vi "Add Bitfile Dialog.vi"(8 "error in (no error)":errorcluster, 11 "Item Ref in":T1 format="%.0x") -> (0 "error out":errorcluster, 1 "RIO Device Address out":string, 2 "Bitfile Path out":path, 3 "Item Ref out":T1 format="%.0x", 5 "OK?":bool)   [LabVIEW 2020, in "Engine Simulation Toolkit System Explorer.lvlib"]
uses:
  Engine Simulation Toolkit System Explorer.lvlib
  <vilib>/NI VeriStand/Custom Device API/Custom Device Item Ref.ctl
  Shared/Properties.vi
  <vilib>/NI VeriStand/Custom Device API/Get Item Property (String Array).vi
  <vilib>/NI VeriStand/Custom Device API/Custom Device API.lvlib
  Shared/Engine Simulation Toolkit Shared.lvlib
panel:
  in  "Warning text":string
  in  "Cancel":bool
  in  "OK":bool
  in  "RIO Device Address":string="RIO0"
  in  "Bitfile Path":path
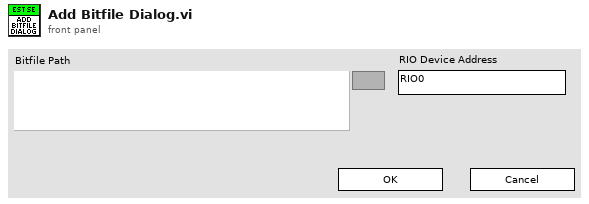
[diagram p1: front panel]
types:
  T1 = typedef "Custom Device API.lvlib/Custom Device Item Ref.ctl" = u64
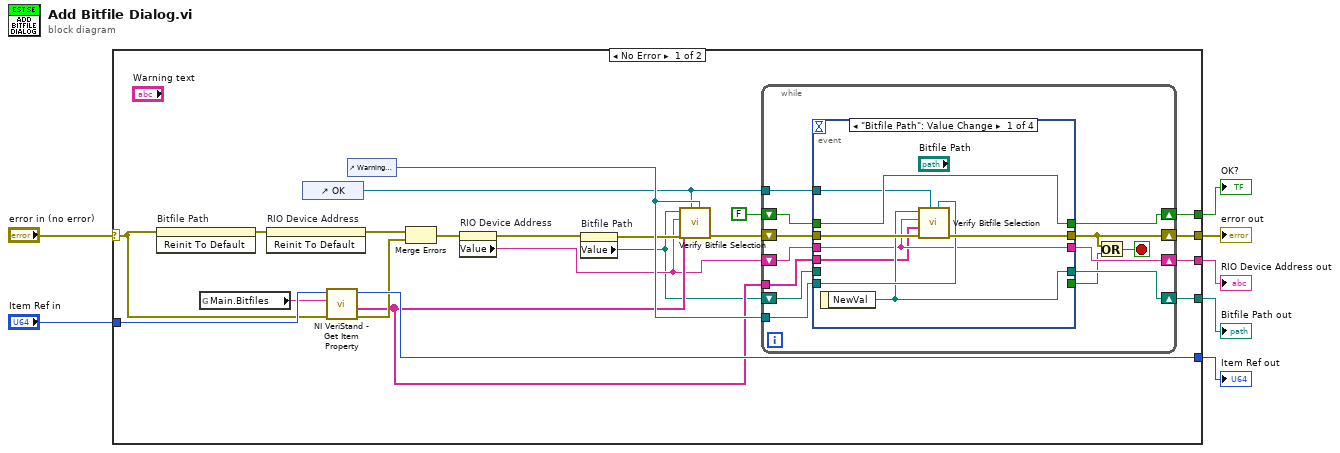
[diagram p0: block diagram]
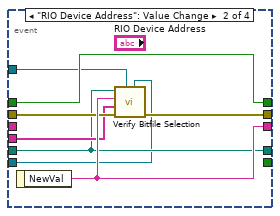
[diagram p2: hidden frame]
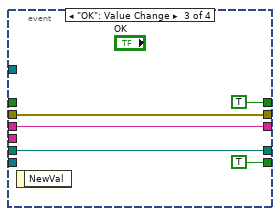
[diagram p3: hidden frame]
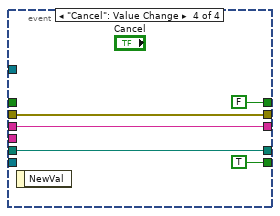
[diagram p4: hidden frame]
diagram:
  n1 = case shown="No Error" "error in (no error)" {
    selector: "error in (no error)" -> [w20 w69]
    tunnel: [w23 w69] -> w7
    tunnel: [w26 _] -> w5
    tunnel: [w25 _] -> w4
    tunnel: [w24 _] -> w3
    tunnel: "Item Ref in" -> [w22 w68]
    tunnel: [w21 w68] -> w1
    frame No Error {
      n2 = invoke on="Bitfile Path" class="Path" method="Reinit To Default"(error in=w20) -> (error out=w28:errorcluster)  [unwired: 2 in, 2 out]
      n3 = global read "Properties.vi" "Main.Bitfiles"() -> (w18:string)
      n4 = invoke on="RIO Device Address" class="Str" method="Reinit To Default"(error in=w28) -> (error out=w8:errorcluster)  [unwired: 2 in, 2 out]
      n5 = control-ref of="OK"() -> (w9:refnum<vi>)
      n6 = call-poly <vilib>:"NI VeriStand - Get Item Property.vi"("error in (no error)"=w20, "Property Name"=w18, "Item Ref in"=w22) -> ("error out"=w19:errorcluster, "Value"=w15:string[], "Item Ref out"=w21:T1)  [unwired: 5 in, 1 out]
      n7 = control-ref of="Warning text"() -> (w16:refnum<vi>)
      n8 = Merge Errors(w8, w19) -> (w14:errorcluster)
      n9 = property on="RIO Device Address" class="Str"(error in=w14) -> (error out=w13:errorcluster, "Value"=w11:string)  [unwired: 1 in, 1 out]
      n10 = property on="Bitfile Path" class="Path"(error in=w13) -> (error out=w12:errorcluster, "Value"=w10:path)  [unwired: 1 in, 1 out]
      n11 = call "Verify Bitfile Selection.vi"("Warning text reference"=w16, "ok button reference in"=w9, "error in (no error)"=w12, "Existing RIO Device Addresses"=w15, "RIO Device Address"=w11, "file path"=w10) -> ("error out"=w17:errorcluster)  [unwired: 5 in]
      n12 = while {
        shift-right: [w39] -> w26
        shift-left: w10 -> [w37]
        shift-right: [w40] -> w25
        shift-left: w11 -> [w38]
        shift-right: [w41] -> w24
        shift-left: FALSE -> [w36]
        tunnel: w9 -> [w35]
        shift-right: [w31] -> w23
        shift-left: w17 -> [w32]
        tunnel: w15 -> [w29]
        tunnel: w16 -> [w30]
        stop <- w34 stop-if-true
        n13 = event shown="[0] \"Bitfile Path\": Value Change" {
          selector: _ -> [_ _ _ _]
          dyn-events: _ -> [_ _ _ _]
          timeout: _ -> [_ _ _ _]
          tunnel: [_ _ TRUE TRUE] -> w33
          tunnel: [w43 w56 w59 w65] -> w40
          tunnel: [w44 w52 w60 w64] -> w39
          tunnel: [w49 w57 TRUE FALSE] -> w41
          tunnel: w38 -> [w43 _ w59 w65]
          tunnel: w37 -> [_ w52 w60 w64]
          tunnel: w36 -> [w49 w57 _ _]
          tunnel: w35 -> [w46 w51 _ _]
          tunnel: w32 -> [w48 w55 w58 w63]
          tunnel: [w47 w54 w58 w63] -> w31
          tunnel: w30 -> [w45 w50 _ _]
          tunnel: w29 -> [w42 w53 _ _]
          event "Bitfile Path": Value Change {
            n14 = event-data() -> ("NewVal"=w44:path)  [unwired: 1 in]
            n15 = call "Verify Bitfile Selection.vi"("Warning text reference"=w45, "ok button reference in"=w46, "error in (no error)"=w48, "Existing RIO Device Addresses"=w42, "RIO Device Address"=w43, "file path"=w44) -> ("error out"=w47:errorcluster)  [unwired: 5 in]
          }
          event "RIO Device Address": Value Change {
            n16 = event-data() -> ("NewVal"=w56:string)  [unwired: 1 in]
            n17 = call "Verify Bitfile Selection.vi"("Warning text reference"=w50, "ok button reference in"=w51, "error in (no error)"=w55, "Existing RIO Device Addresses"=w53, "RIO Device Address"=w56, "file path"=w52) -> ("error out"=w54:errorcluster)  [unwired: 5 in]
          }
          event "OK": Value Change {
            n18 = event-data() -> ()  [unwired: 1 in, 1 out]
          }
          event "Cancel": Value Change {
            n19 = event-data() -> ()  [unwired: 1 in, 1 out]
          }
        }
        n20 = Or(x=w31, y=w33) -> (x .or. y?=w34:bool)
      }
    }
    frame Error {
    }
  }
  "error out" <- w7
  "OK?" <- w3
  "RIO Device Address out" <- w4
  "Bitfile Path out" <- w5
  "Item Ref out" <- w1
